vi "Store Subpanel References.vi"(8 "error in (no error)":errorcluster, 10 "Subpanel References":refnum<vi>[](array[refnum]), 11 "GUI Container in":refnum<class "GUI Container.lvclass">) -> (0 "error out":errorcluster, 2 "Sub Panel Names":string[](array[string]), 3 "GUI Container out":refnum<class "GUI Container.lvclass">)   [LabVIEW 2023, in "GUI Views.lvlib" / "GUI Container.lvclass"]
doc: "This method is used within the \"Actor Core.vi\" of the concrete \"GUI Container\" to store the references of the subpanels present in its front panel and that we want to use as containers."
uses:
  GUI Container.lvclass
  GUI Container.lvclass/GUI Container.ctl
  typedefs/Subpanel Status.ctl
  <vilib>/ErrorRing/Error Ring.xnode
  <vilib>/Utility/error.llb/Error Cluster From Error Code.vi
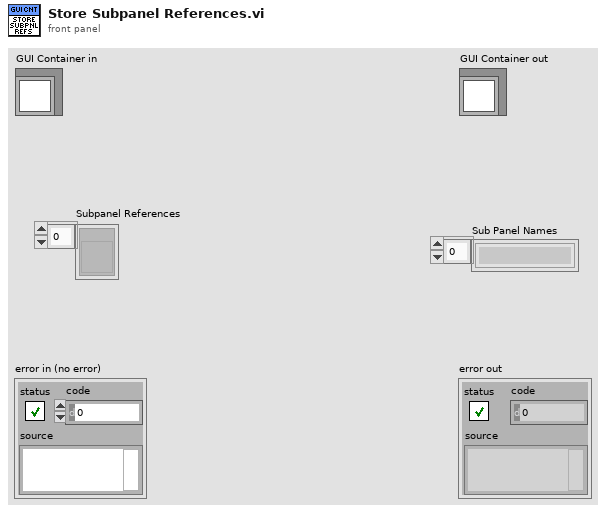
[diagram p1: front panel]
types:
  T1 = typedef "GUI Views.lvlib/GUI Container.lvclass/Subpanel Status.ctl" = cluster{"Subpanel Ref":refnum<vi>, "Inserted View":string, "Inserted View Hierarchy Level":i32}
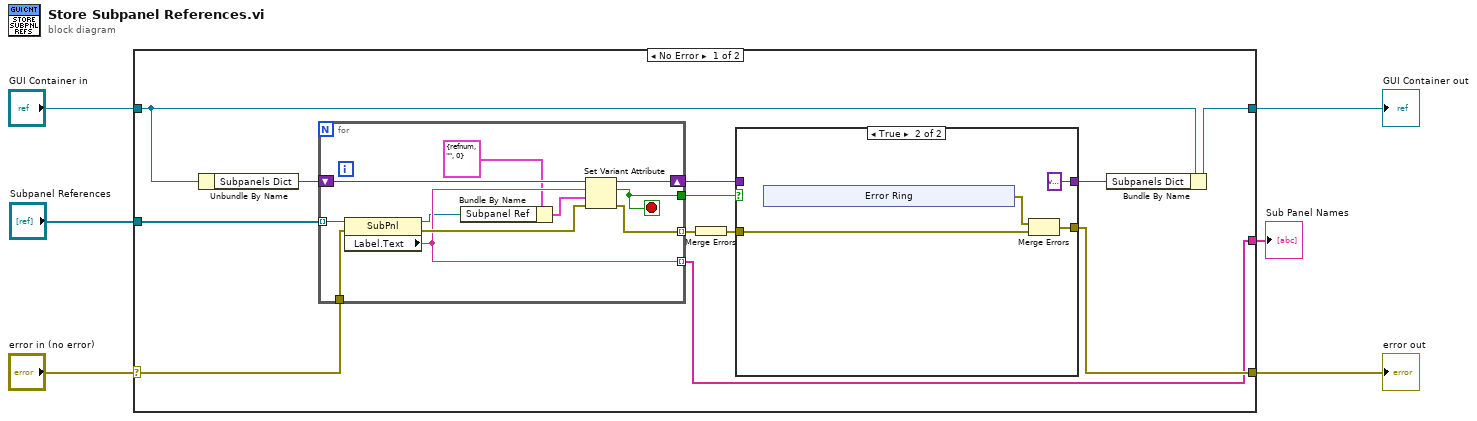
[diagram p0: block diagram]
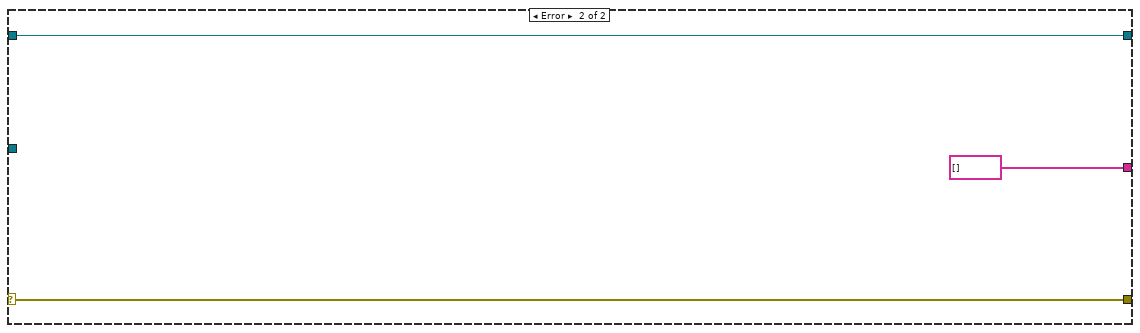
[diagram p3: hidden frame]
diagram:
  n1 = case shown="No Error" "error in (no error)" {
    selector: "error in (no error)" -> [w15 w42]
    tunnel: [w11 w42] -> w5
    tunnel: [w9 w41] -> w3
    tunnel: "GUI Container in" -> [w17 w41]
    tunnel: "Subpanel References" -> [w18 _]
    tunnel: [w7 string[] []] -> w1
    frame No Error {
      n2 = Unbundle By Name(w17) -> ("Subpanels Dict"=w16:variant)
      n3 = for {
        tunnel: w18 -> [w38] mode=indexing
        tunnel: w15 -> [w37]
        tunnel: [w35] -> w14 mode=indexing
        shift-right: [w34] -> w10
        shift-left: w16 -> [w39]
        tunnel: [w33] -> w13
        tunnel: [w32] -> w7 mode=indexing
        stop <- w33 stop-if-true
        n4 = property class="SubPnl"(reference=w38, error in=w37) -> (reference out=w30:refnum<vi>, error out=w36:errorcluster, "Label.Text"=w32:string)
        n5 = Bundle By Name(cluster=T1 {"Subpanel Ref"=refnum, "Inserted View"="", "Inserted View Hierarchy Level"=0} ("Subpanel Status"), "Subpanel Ref"=w30) -> (w29:T1)
        n6 = Set Variant Attribute(Variant=w39, name=w32, value=w29, error in=w36) -> (Variant out=w34:variant, replaced=w33:bool, error out=w35:errorcluster)
      }
      n7 = Merge Errors(w14) -> (w12:errorcluster)
      n8 = case shown="True" w13 {
        tunnel: w12 -> [w20 w21]
        tunnel: [w20 w24] -> w11
        tunnel: w10 -> [w19 _]
        tunnel: [w19 variant ("Subpanels")] -> w8
        frame False {
        }
        frame True {
          n9 = xnode "Error Ring"() -> ("error out"=w22:errorcluster)
          n10 = Merge Errors(w22, w21) -> (w24:errorcluster)
        }
      }
      n11 = Bundle By Name(cluster=w17, "Subpanels Dict"=w8) -> (w9:refnum<class "GUI Container.lvclass">)
    }
    frame Error {
    }
  }
  "error out" <- w5
  "GUI Container out" <- w3
  "Sub Panel Names" <- w1
